vi "Input Parameter Type Definition Name--constant.vi"() -> (3 "Input Parameter Type Definition Name":string)   [LabVIEW 2026]
doc: "This constant defines the name of input parameter type definitions (as a format string)."
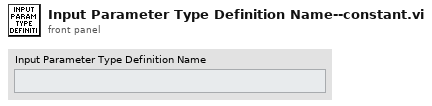
[diagram p1: front panel]
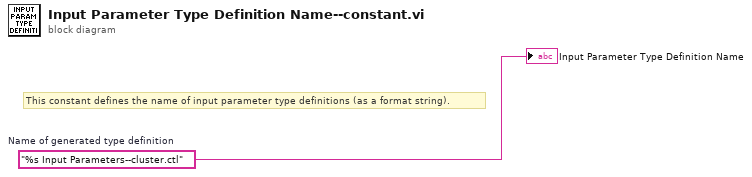
[diagram p0: block diagram]
diagram:
  w1 = "%s Input Parameters--cluster.ctl"  # Name of generated type definition
  # "This constant defines the name of input parameter type definitions (as a format string)."
  "Input Parameter Type Definition Name" <- w1
